vi "editDialog.vi"(0 "reference":refnum<class "NoteNode.lvclass">, 1 "insidePackageNode":bool, 5 "error in (no error)":errorcluster) -> (14 "reference out":refnum<class "NoteNode.lvclass">, 15 "changeConnection":T1, 16 "cancel":bool, 19 "error out":errorcluster)   [LabVIEW 2020, in "NoteNode.lvclass"]
doc: "Edit Dialog"
uses:
  <resource>/Framework/Providers/Open_GDS/UML/NoteNode_class/NoteNode.lvclass
  C:/Program Files (x86)/National Instruments/LabVIEW 2020/resource/Framework/Providers/Open_GDS/UML/RectangularNode_class/RectangularNode.lvclass
  C:/Program Files (x86)/National Instruments/LabVIEW 2020/resource/Framework/Providers/Open_GDS/UML/AbstractNode_class/AbstractNode.lvclass
  <resource>/Framework/Providers/Open_GDS/UML/AbstractNode_class/private/NodeConnectionStatsType.ctl
  <vilib>/Utility/miscctls.llb/LVRectTypeDef.ctl
  <vilib>/event_ctls.llb/eventvkey.ctl
  <resource>/Framework/Providers/Open_GDS/UML/ContextHelp/ContextHelp_HelpTexts.ctl
  <vilib>/Utility/miscctls.llb/LVSelectionTypeDef.ctl
  <resource>/Framework/Providers/Open_GDS/UML/MultiLineString_class/MultiLineString.lvclass
  <resource>/Framework/Providers/Open_GDS/UML/AbstractNode_class/AbstractNode.lvclass
  <resource>/Framework/Providers/Open_GDS/UML/RectangularNode_class/RectangularNode.lvclass
panel:
  in  "Underline":bool
  in  "Italic":bool
  in  "Bold":bool
  in  "Justify":u16(ring) items=["Left", "Center", "Right"]
  in  "Note color":u32(colorbox)
  in  "Help":bool
  in  "TextBox":string
  in  "connection":bool caption="Connect to Package"
  in  "OK Button":bool
  in  "Cancel Button":bool
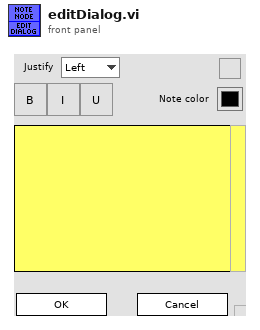
[diagram p1: front panel]
types:
  T1 = typedef "AbstractNode.lvclass/NodeConnectionStatsType.ctl" = enum16{"NA", "Connect", "DisConnect"}
  T2 = typedef "LVRectTypeDef.ctl" = cluster{"Left":i16, "Top":i16, "Right":i16, "Bottom":i16}
  T3 = cluster{"IgnoreStyleUpdate":bool, "Text":string, "Cancelled":bool, "InitSize":T2, "WidthChanged":bool}
  T4 = typedef "ContextHelp_HelpTexts.ctl" = enum16{"None(Hide)", "Default", "Help", "Welcome", "GettingStarted", "ClassDiagram_Help", "SequenceDiagram_Help", "UseCaseDiagram_Help", "BSelect", "BClass", "BInterface", "BPackage", "BNote", "BDependency", "BInheritance", "BInterfaceImplementation", "BAssociation", "BAggregation", "BCompAggregation", "BNoteConnector", "BObject", "BActionBar", "BCall", "BSystem", "BActor", "BUseCase", "BGeneralization", "BIncludes", "BExtends", "BUseCaseDiagramAssociation", "ClassRelationshipEdge editDialog_Bent Style", "ClassRelationshipEdge editDialog_RelationType", "ClassRelationshipEdge editDialog_Reverse association", "ClassRelationshipEdge editDialog_Start label", "ClassRelationshipEdge editDialog_Middle label", "ClassRelationshipEdge editDialog_End label", "UMLEditor reversedEngineering_Pathes", "ReversedEngineering StateReverseDialog_Help", "ReversedEngineering StateQueuedSettings_Help", "UMLEditor reversedEngineering_AddTopVIs", "UMLEditor reversedEngineering_AddClasses", "UMLEditor reversedEngineering_AddDirs", "UMLEditor reversedEngineering_Recursively", "UMLEditor reversedEngineering_Remove", "UMLEditor reversedEngineering_ClearList", "UMLEditor reversedEngineering_HideSubAss", "UMLEditor reversedEngineering_CreateTypes", "UMLEditor reversedEngineering_OnlyInheritance", "UMLEditor reversedEngineering_CreateApplication", "UMLEditor reversedEngineering_OK", "UMLEditor reversedEngineering_Cancel", "UMLEditor reversedEngineering_Help", "UMLEditor createWizardScriptFile_ScriptfilePath", "UMLEditor createWizardScriptFile_ClassPath", "UMLEditor createWizardScriptFile_Use", "UMLEditor createWizardScriptFile_PrivateDirName", "UMLEditor createWizardScriptFile_DirAppend", "UMLEditor createWizardScriptFile_Separator Character", "UMLEditor createWizardScriptFile_OK", "UMLEditor createWizardScriptFile_Cancel", "UMLEditor createWizardScriptFile_Help", "ClassNode editDialog_Class Name", "InterfaceNode editDialog_Class Name", "ClassNode editDialog_Attribute", "ClassNode editDialog_Methods", "InterfaceNode editDialog_Methods", "ClassNode editDialog_connection", "InterfaceNode editDialog_connection", "ClassNode editDialog_StereoType", "ClassNode editDialog_ShowAttrib", "ClassNode editDialog_ShowMethods", "ClassNode editDialog_ClassPath", "ClassNode editDialog_AddAttribute", "ClassNode editDialog_AddMethod", "InterfaceNode editDialog_AddMethod", "ClassNode AttributeGuide_AttributeName", "ClassNode AttributeGuide_Array?", "ClassNode AttributeGuide_Data Type", "ClassNode AttributeGuide_RefName", "ClassNode AttributeGuide_Preview", "ClassNode AttributeGuide_OK", "ClassNode AttributeGuide_Cancel", "ClassNode MethodGuide_Visibility", "ClassNode MethodGuide_Method Name", "ClassNode MethodGuide_Preview", "ClassNode MethodGuide_OK", "ClassNode MethodGuide_Cancel", "CallNode EditCallProperties_AllButtons", "ObjectNode EditObjectlProperties_AllButtons", "ActorNode EditActorProperties_AllButtons", "UseCaseRelationshipNode EditUseCaselProperties_AllButtons", "UseCaseNode EditUseCaselProperties_AllButtons", "SystemNode EditSystemProperties_AllButtons", "ReversedEngineering UpdateAttributes_AllButtons", "StateNode editDialog_AllButtons", "StateTransition editDialog_AllButtons", "ArrangeNodes Main_Picture", "ArrangeNodes Main_Zoom", "ArrangeNodes Main_Auto Zoom", "ArrangeNodes Main_shorten", "ArrangeNodes Main_Min Length", "ArrangeNodes Main_Max Length", "ArrangeNodes Main_increase", "ArrangeNodes Main_decrease", "ArrangeNodes Main_Shake", "ArrangeNodes Main", "BState", "BInitialState", "BFinalState", "BStateTransition", "StateDiagram_Help", "StateDiagram_PropertiesAllButtons", "ReversedEngineering StateReverseDialog_ClearStates", "ReversedEngineering StateReverseDialog_UseQueuedStateMachines", "ReversedEngineering StateReverseDialog_QueuedSettings", "ReversedEngineering StateReverseDialog_SearchForVIs", "ReversedEngineering StateReverseDialog_SearchCriteria", "OptionsDialog_ClassBasePath", "OptionsDialog_VIPath", "OptionsDialog_ApplicationPath", "OptionsDialog_WizDir", "OptionsDialog_IniFilePath", "OptionsDialog_DefineColors", "OptionsDialog_Help", "OptionsDialog_CreateTypes", "ClassRelationshipEdge editDialog_SplitWire"}
  T5 = typedef "LVSelectionTypeDef.ctl" = cluster{"Selection Start":u32, "Selection End":u32}
  T6 = typedef "NoteNode.lvclass/ObjectAttributes.ctl" = cluster{"DEFAULT_WIDTH":i32, "DEFAULT_HEIGHT":i32, "DEFAULT_COLOR":u32, "FOLD_X":i32, "FOLD_Y":i32, "color":u32, "text":refnum<class "MultiLineString.lvclass">, "pointNodes":refnum<class "AbstractNode.lvclass">[]}
  T7 = typedef "RectangularNode.lvclass/ObjectAttributes.ctl" = cluster{"bounds":T8}
  T8 = typedef "Rectangle Rectangle2D.ctl" = cluster{"x":dbl, "y":dbl, "width":dbl, "height":dbl}
  T9 = typedef "AbstractNode.lvclass/ObjectAttributes.ctl" = cluster{"parent":refnum<class "AbstractNode.lvclass">, "children":refnum<class "AbstractNode.lvclass">[], "Hidden":bool}
  T10 = typedef "MultiLineString.lvclass/JustificationType.ctl" = enum16{"LEFT", "CENTER", "RIGHT"}
  T11 = typedef "eventvkey.ctl" = enum16{"ASCII", "Enter", "Return", "Shift", "Ctrl", "Alt", "Cmd", "Opt", "Caps", "NumLock", "Clear", "Break", "Up", "Down", "Left", "Right", "Insert", "Delete", "Home", "End", "PageUp", "PageDown", "Escape", "Help", "Pause", "ScrollLock", "F1", "F2", "F3", "F4", "F5", "F6", "F7", "F8", "F9", "F10", "F11", "F12", "F13", "F14", "F15", "F16", "F17", "F18", "F19", "F20", "F21", "F22", "F23", "F24", "Play", "VolumeUp", "VolumeDown", "Mute", "Two Byte Char"}
  T12 = cluster{"Shift":bool, "Ctrl":bool, "Alt":bool, "Cmd":bool, "Opt":bool}
  T13 = typedef "ContextHelp_ShowType.ctl" = cluster{"Header":string, "Picture":picture, "Text":string}
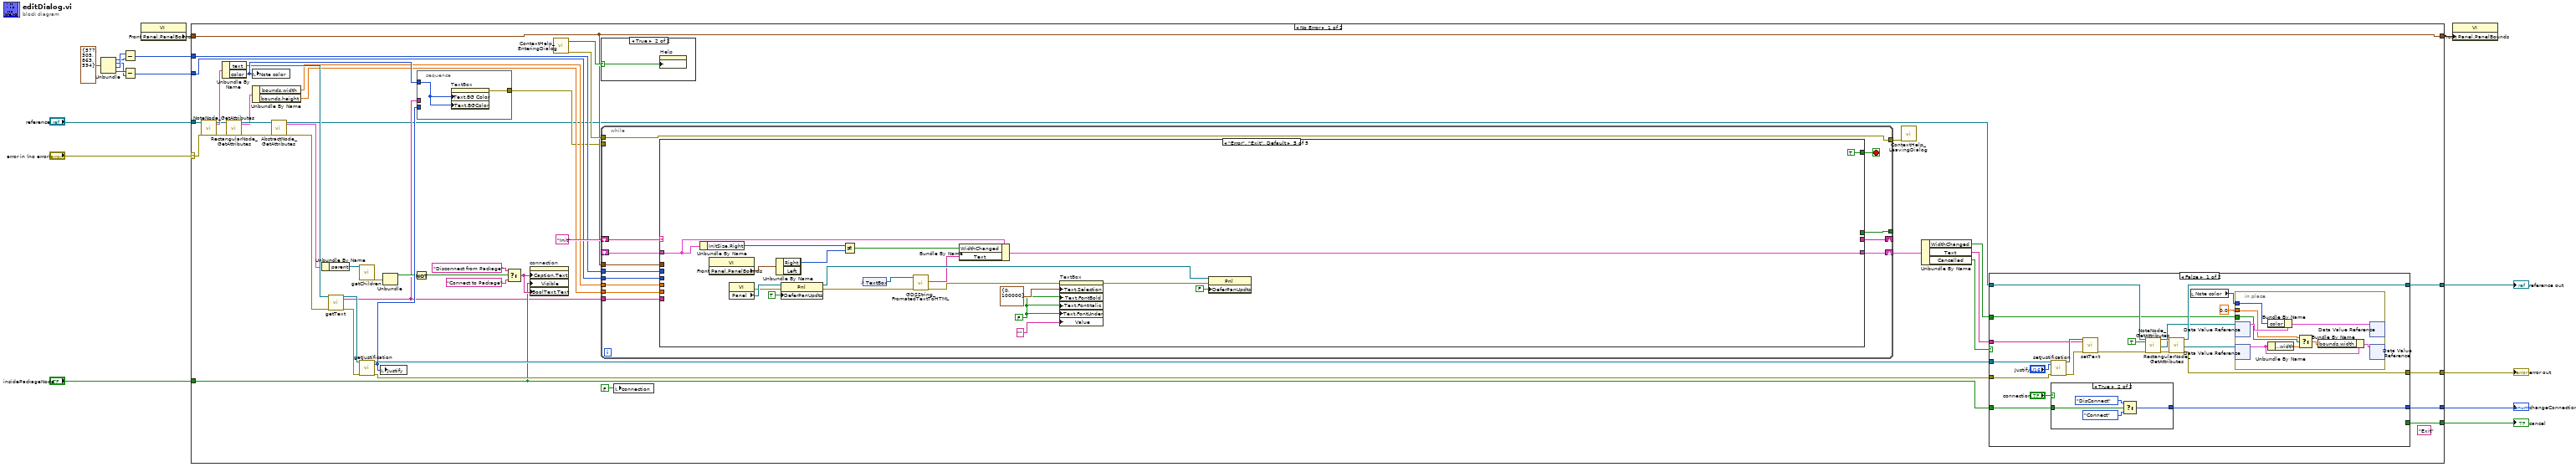
[diagram p0: block diagram]
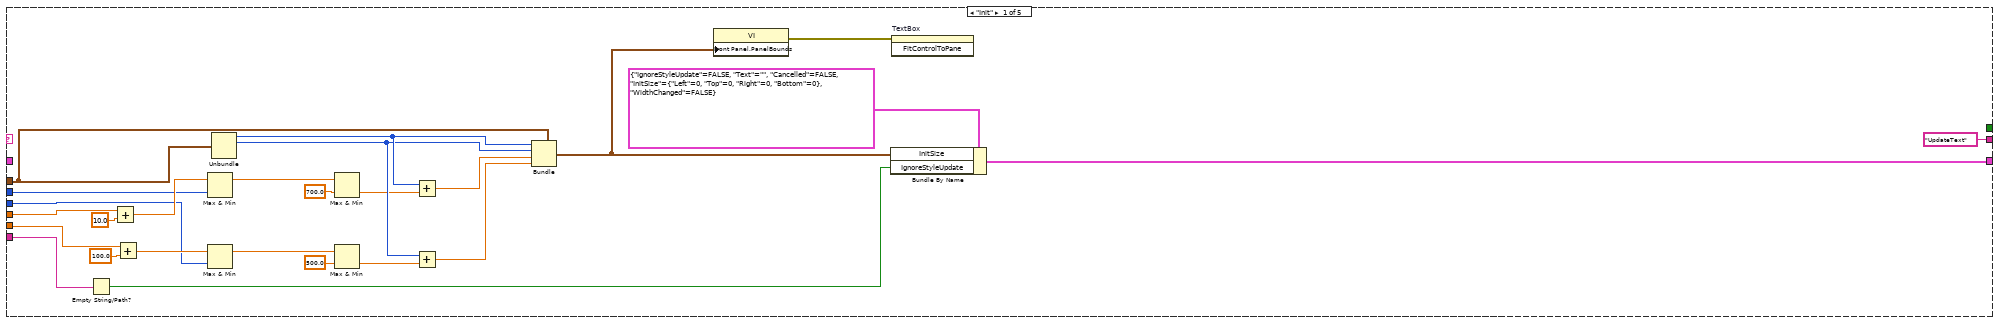
[diagram p3: hidden frame]
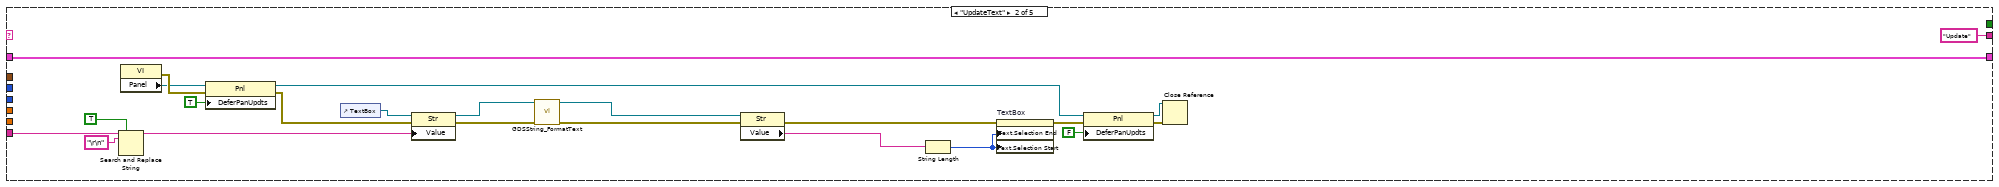
[diagram p4: hidden frame]
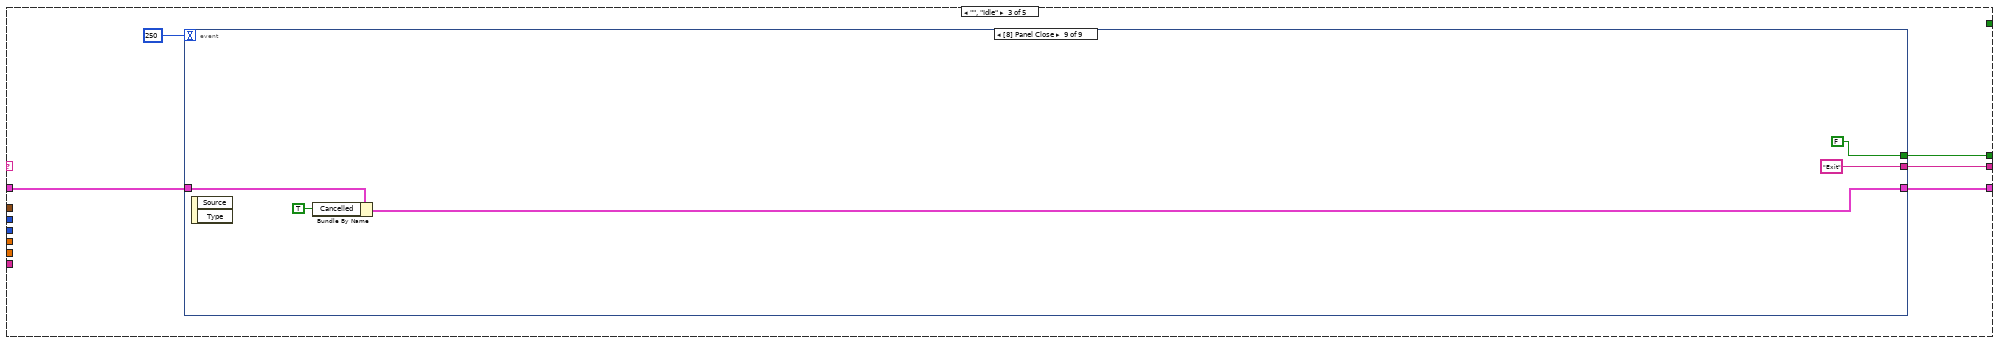
[diagram p5: hidden frame]
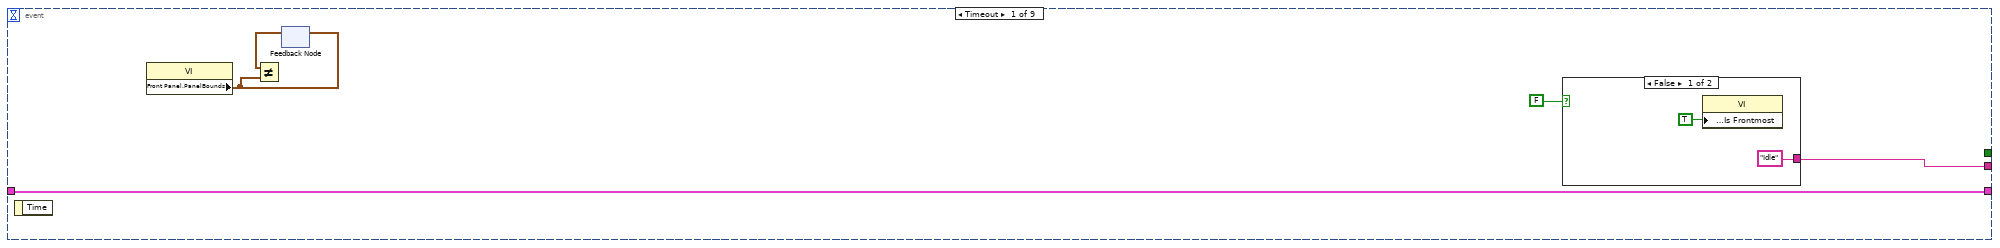
[diagram p6: hidden frame]
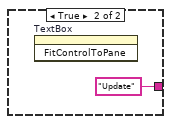
[diagram p7: hidden frame]
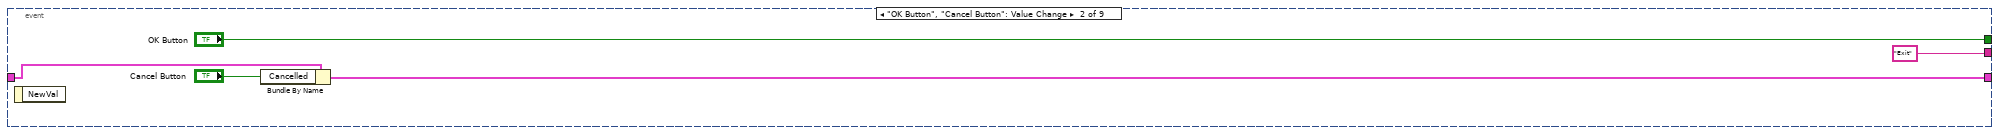
[diagram p8: hidden frame]
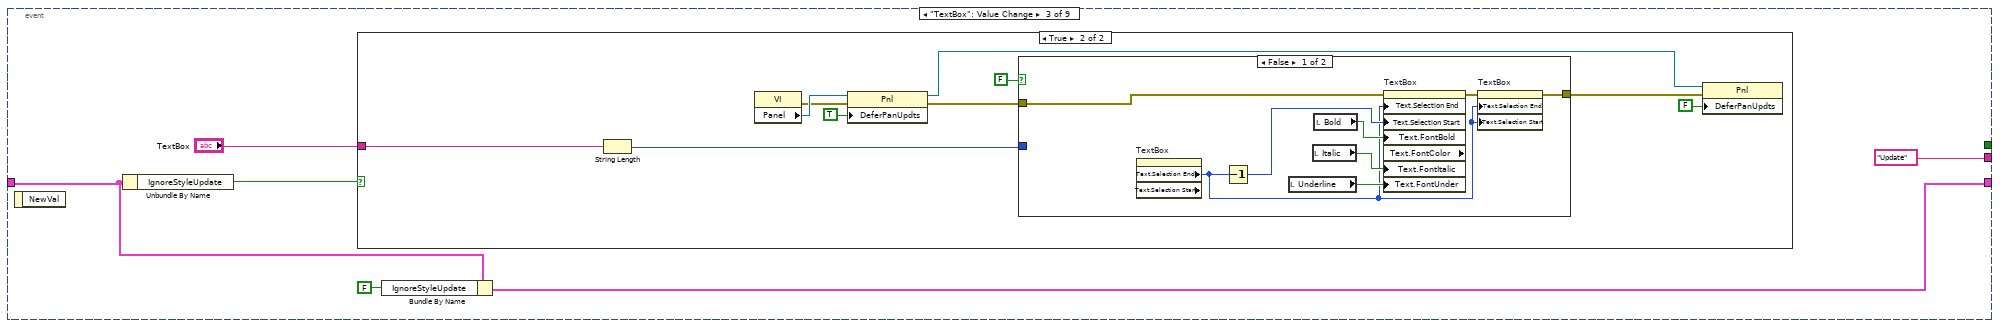
[diagram p9: hidden frame]
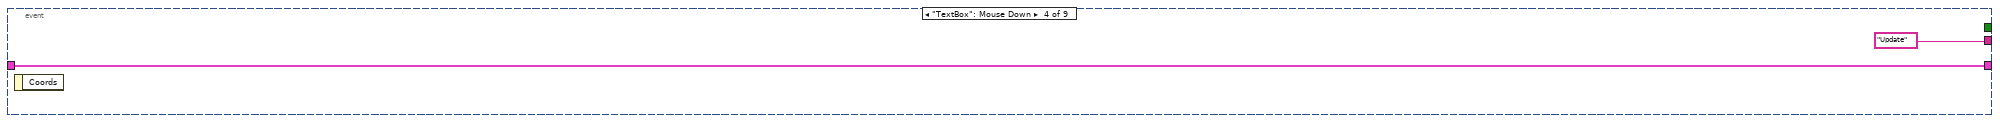
[diagram p12: hidden frame]
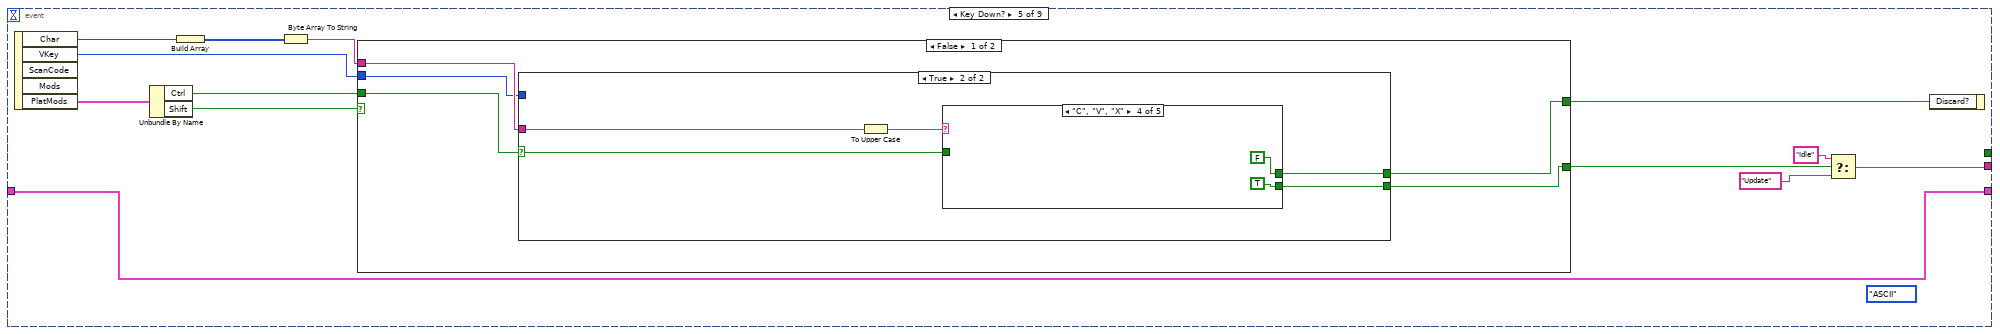
[diagram p13: hidden frame]
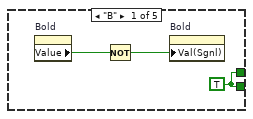
[diagram p16: hidden frame]
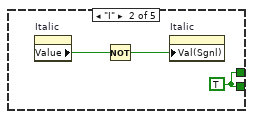
[diagram p17: hidden frame]
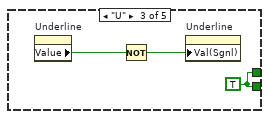
[diagram p18: hidden frame]
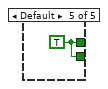
[diagram p19: hidden frame]
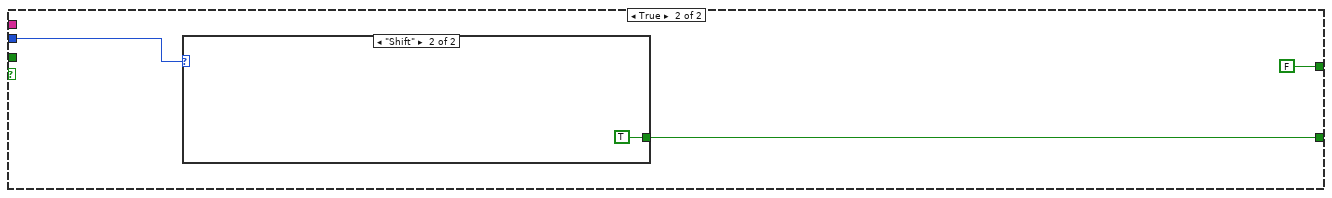
[diagram p20: hidden frame]
diagram:
  n1 = Unbundle(T2 {"Left"=577, "Top"=305, "Right"=863, "Bottom"=594} ("Front Panel Window:Panel Bounds")) -> ("Left"=w6:i16, "Top"=w4:i16, "Right"=w7:i16, "Bottom"=w5:i16)
  n2 = Subtract(x=w7, y=w6) -> (x-y=w2:i16)
  n3 = Subtract(x=w5, y=w4) -> (x-y=w1:i16)
  n4 = property class="VI"() -> ("Front Panel.PanelBounds"=w9:T2)  [unwired: 2 in, 2 out]
  n5 = case shown="No Error" "error in (no error)" {
    selector: "error in (no error)" -> [w58 w349]
    tunnel: "reference" -> [w59 w350]
    tunnel: [w62 w349] -> w14
    tunnel: [w61 w350] -> w13
    tunnel: [w56 TRUE ("Key Focus")] -> w12
    tunnel: [w47 _] -> w11
    tunnel: "insidePackageNode" -> [w39 _]
    tunnel: w9 -> [w29 w347]
    tunnel: [w29 w347] -> w3
    tunnel: w2 -> [w31 _]
    tunnel: w1 -> [w30 _]
    frame No Error {
      (unwired) "Exit"
      n6 = call <resource>:"NoteNode_GetAttributes.vi"("reference in"=w59, "error in (no error)"=w58) -> ("reference out"=w24:refnum<class "NoteNode.lvclass">, "Data"=w25:T6, "error out"=w23:errorcluster)  [unwired: 1 in, 14 out]
      n7 = Unbundle By Name(w25) -> ("text"=w57:refnum<class "MultiLineString.lvclass">, "color"=w60:u32)
      n8 = call <resource>:"RectangularNode_GetAttributes.vi"("reference in"=w24, "error in (no error)"=w23) -> ("reference out"=w22:refnum<class "NoteNode.lvclass">, "Data"=w17:T7, "error out"=w21:errorcluster)  [unwired: 14 in, 1 out]
      n9 = local write "Note color"(w60) -> ()
      n10 = Unbundle By Name(w17) -> ("bounds.width"=w33:dbl, "bounds.height"=w32:dbl)
      n11 = call <resource>:"AbstractNode_GetAttributes.vi"("reference in"=w22, "error in (no error)"=w21) -> ("reference out"=w19:refnum<class "NoteNode.lvclass">, "Data"=w18:T9, "error out"=w20:errorcluster)  [unwired: 14 in, 1 out]
      n12 = Unbundle By Name(w18) -> ("parent"=w44:refnum<class "AbstractNode.lvclass">)
      n13 = call-dynamic "getText.vi"("reference"=w57, "error in (no error)"=w20) -> ("reference out"=w52:refnum<class "MultiLineString.lvclass">, "text"=w36:string, "error out"=w51:errorcluster)  [unwired: 15 in]
      n14 = call-dynamic "getChildren.vi"("reference"=w44) -> ("error out"=w42:errorcluster)  [unwired: 15 in, 3 out]
      n15 = call <resource>:"getJustification.vi"("reference"=w52, "error in (no error)"=w51) -> ("reference out"=w49:refnum<class "MultiLineString.lvclass">, "justification"=w48:T10, "error out"=w50:errorcluster)  [unwired: 15 out]
      n16 = local write "Justify"(w48) -> ()
      n17 = Unbundle(w42) -> ("status"=w43:bool)  [unwired: 2 out]
      n18 = Not(x=w43) -> (.not. x?=w45:bool)
      n19 = stacked-sequence {
        tunnel: w60 -> [w346]
        tunnel: w36 -> [_]
        tunnel: w48 -> [_]
        tunnel: [w345] -> w28
        frame #0 {
          n20 = property on="TextBox" class="Str"("Text.BG Color"=w346, "Text.BGColor"=w346) -> (error out=w345:errorcluster)  [unwired: 2 in, 1 out]
        }
      }
      n21 = Select(t="Disconnect from Package", s=w45, f="Connect to Package") -> (s? t:f=w46:string)
      n22 = property on="connection" class="Bool (strict)"("Caption.Text"=w46, "Visible"=w39, "BoolText.Text"=w46) -> ()  [unwired: 2 in, 2 out]
      n23 = call <resource>:"ContextHelp_EnteringDialog.vi"() -> ("HelpStatus"=w53:bool, "error out"=w54:errorcluster)  [unwired: 3 in, 15 out]
      n24 = case shown="True" w53 {
        selector: w53 -> [_ w63]
        frame False {
        }
        frame True {
          n25 = property on="Help" class="Bool (strict)"("Value (Signaling)"=w63) -> ()  [unwired: 2 in, 2 out]
        }
      }
      n26 = while {
        tunnel: [w76] -> _
        tunnel: [w74] -> w55
        tunnel: w54 -> [w74]
        shift-right: [w71] -> _
        shift-left: "Init" -> [w73]
        tunnel: w36 -> [w72]
        shift-right: [w70] -> w35
        shift-left: _ -> [w69]
        tunnel: w33 -> [w68]
        tunnel: w32 -> [w67]
        tunnel: w31 -> [w66]
        tunnel: w30 -> [w65]
        tunnel: w29 -> [w64]
        tunnel: w28 -> [_]
        stop <- w75 stop-if-true
        n27 = case shown="\"Error\", \"Exit\", Default" w73 {
          tunnel: [_ _ w130 _ _] -> w76
          tunnel: [_ _ _ _ TRUE ("Key Focus")] -> w75
          tunnel: w72 -> [w82 w107 _ _ _]
          tunnel: ["UpdateText" "Update" w128 _ _] -> w71
          tunnel: [w79 w116 w126 w239 w292] -> w70
          tunnel: w69 -> [_ w116 w127 w240 w291]
          tunnel: w68 -> [w101 _ _ _ _]
          tunnel: w67 -> [w100 _ _ _ _]
          tunnel: w66 -> [w95 _ _ _ _]
          tunnel: w65 -> [w94 _ _ _ _]
          tunnel: w64 -> [w93 _ _ _ _]
          frame "Init" {
            n28 = Empty String/Path?(string/path=w82) -> (empty?=w80:bool)
            n29 = Add(x=w101, y=10.0) -> (x+y=w97:dbl)
            n30 = Add(x=w100, y=100.0) -> (x+y=w96:dbl)
            n31 = Max & Min(x=w97, y=w95) -> (max(x,y)=w86:dbl)  [unwired: 1 out]
            n32 = Max & Min(x=w96, y=w94) -> (max(x,y)=w88:dbl)  [unwired: 1 out]
            n33 = Unbundle(w93) -> ("Left"=w92:i16, "Top"=w90:i16)  [unwired: 2 out]
            n34 = Max & Min(x=w86, y=700.0) -> (min(x,y)=w85:dbl)  [unwired: 1 out]
            n35 = Max & Min(x=w88, y=500.0) -> (min(x,y)=w87:dbl)  [unwired: 1 out]
            n36 = Add(x=w92, y=w85) -> (x+y=w91:dbl)
            n37 = Add(x=w90, y=w87) -> (x+y=w89:dbl)
            n38 = Bundle(cluster=w93, "Left"=w92, "Top"=w90, "Right"=w91, "Bottom"=w89) -> (w77:T2)
            n39 = property class="VI"("Front Panel.PanelBounds"=w77) -> (error out=w78:errorcluster)  [unwired: 2 in, 1 out]
            n40 = Bundle By Name(cluster=T3 {"IgnoreStyleUpdate"=FALSE, "Text"="", "Cancelled"=FALSE, "InitSize"={"Left"=0, "Top"=0, "Right"=0, "Bottom"=0}, "WidthChanged"=FALSE} ("State"), "InitSize"=w77, "IgnoreStyleUpdate"=w80) -> (w79:T3)
            n41 = invoke on="TextBox" class="Str" method="FitControlToPane"(error in=w78) -> ()  [unwired: 2 in, 3 out]
          }
          frame "UpdateText" {
            n42 = Search and Replace String(replace all?=TRUE ("replace all? (F)"), input string=w107, search string="\r\n") -> (result string=w106:string)  [unwired: 5 in, 3 out]
            n43 = property class="VI"() -> (error out=w121:errorcluster, "Panel"=w119:refnum<vi>)  [unwired: 2 in, 1 out]
            n44 = property class="Pnl"(reference=w119, error in=w121, "DeferPanUpdts"=TRUE ("Defer Panel Updates")) -> (reference out=w123:refnum<vi>, error out=w122:errorcluster)
            n45 = control-ref of="TextBox"() -> (w115:refnum<vi>)
            n46 = property on="Property Node" class="Str"(reference=w115, error in=w122, "Value"=w106) -> (reference out=w117:refnum<vi>, error out=w118:errorcluster)
            n47 = call <resource>:"GDSString_FormatText.vi"("TextIn"=w117, "error in"=w118) -> ("TextOut"=w114:refnum<vi>, "error out"=w113:errorcluster)  [unwired: 16 in]
            n48 = property on="Property Node" class="Str"(reference=w114, error in=w113) -> (error out=w112:errorcluster, "Value"=w111:string)  [unwired: 1 out]
            n49 = String Length(string=w111) -> (length=w108:i32)
            n50 = property on="TextBox" class="Str"(error in=w112, "Text.Selection End"=w108, "Text.Selection Start"=w108) -> (error out=w110:errorcluster)  [unwired: 1 in, 1 out]
            n51 = property class="Pnl"(reference=w123, error in=w110, "DeferPanUpdts"=FALSE ("Defer Panel Updates")) -> (reference out=w124:refnum<vi>, error out=w105:errorcluster)
            n52 = Close Reference(reference=w124, error in (no error)=w105) -> ()  [unwired: 1 out]
          }
          frame "", "Idle" {
            n53 = event shown="[8] Panel Close" {
              selector: _ -> [_ _ _ _ _ _ _ _ _]
              dyn-events: _ -> [_ _ _ _ _ _ _ _ _]
              timeout: 250 -> [_ _ _ _ _ _ _ _ _]
              tunnel: [_ "OK Button" _ _ _ _ _ _ FALSE ("OK Button")] -> w130
              tunnel: [w132 "Exit" "Update" "Update" w171 _ "Update" "Idle" "Exit"] -> w128
              tunnel: w127 -> [w135 w141 w146 w170 w183 w212 w218 w227 w236]
              tunnel: [w135 w140 w147 w170 w183 w212 w217 w227 w235] -> w126
              event Timeout {
                n54 = event-data() -> ()  [unwired: 2 out]
                n55 = property class="VI"() -> ("Front Panel.PanelBounds"=w134:T2)  [unwired: 2 in, 2 out]
                n56 = feedback-in #1(w134) -> ()
                n57 = feedback #1() -> (w133:T2)  [unwired: 1 in]
                n58 = Not Equal?(x=w133, y=w134) -> ()  [unwired: 1 out]
                n59 = case shown="False" FALSE {
                  tunnel: ["Idle" "Update"] -> w132
                  frame False {
                    n60 = property class="VI"("Front Panel Window:Is Frontmost"=TRUE) -> ()  [unwired: 2 in, 2 out]
                  }
                  frame True {
                    n61 = invoke on="TextBox" class="Str" method="FitControlToPane"() -> ()  [unwired: 3 in, 3 out]
                  }
                }
              }
              event "OK Button", "Cancel Button": Value Change {
                n62 = event-data() -> ()  [unwired: 2 out]
                n63 = Bundle By Name(cluster=w141, "Cancelled"="Cancel Button") -> (w140:T3)
              }
              event "TextBox": Value Change {
                n64 = event-data() -> ()  [unwired: 2 out]
                n65 = Unbundle By Name(w146) -> ("IgnoreStyleUpdate"=w149:bool)
                n66 = case shown="True" w149 {
                  tunnel: "TextBox" -> [_ w151]
                  frame False {
                  }
                  frame True {
                    n67 = String Length(string=w151) -> (length=w152:i32)
                    n68 = property class="VI"() -> (error out=w157:errorcluster, "Panel"=w159:refnum<vi>)  [unwired: 2 in, 1 out]
                    n69 = property class="Pnl"(reference=w159, error in=w157, "DeferPanUpdts"=TRUE ("Defer Panel Updates")) -> (reference out=w155:refnum<vi>, error out=w154:errorcluster)
                    n70 = case shown="False" FALSE {
                      tunnel: w152 -> [_ _]
                      tunnel: w154 -> [w166 w168]
                      tunnel: [w164 w168] -> w153
                      frame False {
                        n71 = property on="TextBox" class="Str" props=["Text", "Selection End", "Text", "Selection Start"]() -> ("Text.Selection End"=w160:u32)  [unwired: 2 in, 3 out]
                        n72 = Decrement(x=w160) -> (x-1=w167:u32)
                        n73 = local read "Underline"() -> (w161:bool)
                        n74 = local read "Italic"() -> (w162:bool)
                        n75 = local read "Bold"() -> (w163:bool)
                        n76 = property on="TextBox" class="Str" props=["Text", "Selection End", "Text", "Selection Start", "Text", "FontBold", "Text", "FontColor", "Text", "FontItalic", "Text", "FontUnder"](error in=w166, "Text.Selection End"=w160, "Text.Selection Start"=w167, "Text.FontBold"=w163, "Text.FontItalic"=w162, "Text.FontUnder"=w161) -> (error out=w165:errorcluster)  [unwired: 1 in, 2 out]
                        n77 = property on="TextBox" class="Str"(error in=w165, "Text.Selection End"=w160, "Text.Selection Start"=w160) -> (error out=w164:errorcluster)  [unwired: 1 in, 1 out]
                      }
                      frame True {
                      }
                    }
                    n78 = property class="Pnl"(reference=w155, error in=w153, "DeferPanUpdts"=FALSE ("Defer Panel Updates")) -> ()  [unwired: 2 out]
                  }
                }
                n79 = Bundle By Name(cluster=w146, "IgnoreStyleUpdate"=FALSE ("NewType")) -> (w147:T3)
              }
              event "TextBox": Mouse Down {
                n80 = event-data() -> ()  [unwired: 2 out]
              }
              event Key Down? {
                (unwired) eventvkey."ASCII" ("VKey")
                n81 = event-data() -> ("Char"=w178:i16, "VKey"=w177:T11, "PlatMods"=w176:T12)  [unwired: 3 out]
                n82 = Unbundle By Name(w176) -> ("Ctrl"=w180:bool, "Shift"=w179:bool)
                n83 = Build Array(w178) -> (w182:i16[])
                n84 = Byte Array To String(unsigned byte array=w182) -> (string=w181:string)
                n85 = case shown="False" w179 {
                  tunnel: w180 -> [w188 _]
                  tunnel: w181 -> [w187 _]
                  tunnel: [w186 FALSE ("Discard?")] -> w175
                  tunnel: [w185 w209] -> w174
                  tunnel: w177 -> [w184 w207]
                  frame False {
                    n86 = case shown="True" w188 {
                      selector: w188 -> [_ w192]
                      tunnel: w187 -> [_ w194]
                      tunnel: [_ w191] -> w186
                      tunnel: [_ w190] -> w185
                      tunnel: w184 -> [w189 _]
                      frame False {
                        n87 = case shown="\"ASCII\", Default" w189 {
                          frame "ASCII", Default {
                          }
                          frame "Home" {
                          }
                        }
                      }
                      frame True {
                        n88 = To Upper Case(1:w194) -> (0:w193:string)
                        n89 = case shown="\"C\", \"V\", \"X\"" w193 {
                          tunnel: w192 -> [_ _ _ _ _]
                          tunnel: [w195 w198 w201 FALSE ("Discard?") w206] -> w191
                          tunnel: [w195 w198 w201 TRUE ("Discard?") w206] -> w190
                          frame "B" {
                            w195 = TRUE ("Discard?")
                            n90 = property on="Bold" class="Bool (strict)"() -> ("Value"=w197:bool)  [unwired: 2 in, 2 out]
                            n91 = Not(x=w197) -> (.not. x?=w196:bool)
                            n92 = property on="Bold" class="Bool (strict)"("Val(Sgnl)"=w196) -> ()  [unwired: 2 in, 2 out]
                          }
                          frame "I" {
                            w198 = TRUE ("Discard?")
                            n93 = property on="Italic" class="Bool (strict)"() -> ("Value"=w200:bool)  [unwired: 2 in, 2 out]
                            n94 = Not(x=w200) -> (.not. x?=w199:bool)
                            n95 = property on="Italic" class="Bool (strict)"("Val(Sgnl)"=w199) -> ()  [unwired: 2 in, 2 out]
                          }
                          frame "U" {
                            w201 = TRUE ("Discard?")
                            n96 = property on="Underline" class="Bool (strict)"() -> ("Value"=w203:bool)  [unwired: 2 in, 2 out]
                            n97 = Not(x=w203) -> (.not. x?=w202:bool)
                            n98 = property on="Underline" class="Bool (strict)"("Val(Sgnl)"=w202) -> ()  [unwired: 2 in, 2 out]
                          }
                          frame "C", "V", "X" {
                          }
                          frame Default {
                            w206 = TRUE
                          }
                        }
                      }
                    }
                  }
                  frame True {
                    n99 = case shown="\"Shift\"" w207 {
                      tunnel: [_ TRUE] -> w209
                      frame Default {
                      }
                      frame "Shift" {
                      }
                    }
                  }
                }
                n100 = Select(t="Idle", s=w174, f="Update") -> (s? t:f=w171:string)
                n101 = event-data("Discard?"=w175) -> ()  [unwired: 1 in, 1 out]
              }
              event "Note color": Value Change {
                (unwired) "Idle"
                n102 = event-data() -> ()  [unwired: 2 out]
                n103 = property on="TextBox" class="Str"("Text.BG Color"="Note color", "Text.BGColor"="Note color") -> ()  [unwired: 2 in, 2 out]
              }
              event "Bold", "Italic", "Underline": Value Change {
                (unwired) TRUE ("Data Changed?")
                n104 = event-data() -> ()  [unwired: 2 out]
                n105 = property on="TextBox" class="Str"() -> ("Text.Selection End"=w223:u32, "Text.Selection Start"=w222:u32)  [unwired: 2 in, 2 out]
                n106 = local read "TextBox"() -> (w221:string)
                n107 = String Length(string=w221) -> (length=w220:i32)
                n108 = Equal?(x=w223, y=w222) -> (x = y?=w219:bool)
                n109 = Bundle By Name(cluster=w218, "IgnoreStyleUpdate"=w219) -> (w217:T3)
                n110 = case shown="False" w219 {
                  tunnel: "Bold" -> [w226 _]
                  tunnel: w220 -> [_ _]
                  tunnel: "Italic" -> [w225 _]
                  tunnel: "Underline" -> [w224 _]
                  frame False {
                    n111 = property on="TextBox" class="Str"("Text.FontUnder"=w224) -> ()  [unwired: 2 in, 2 out]
                    n112 = property on="TextBox" class="Str"("Text.FontBold"=w226) -> ()  [unwired: 2 in, 2 out]
                    n113 = property on="TextBox" class="Str"("Text.FontItalic"=w225) -> ()  [unwired: 2 in, 2 out]
                  }
                  frame True {
                  }
                }
              }
              event "Help": Value Change {
                n114 = event-data() -> ()  [unwired: 2 out]
                n115 = case shown="True" "Help" {
                  tunnel: [ContextHelp_HelpTexts."None(Hide)" ("HelpText") ContextHelp_HelpTexts."BNote" ("HelpText")] -> w230
                  frame False {
                  }
                  frame True {
                  }
                }
                n116 = call <resource>:"ContextHelp_HelpTexts.vi"("HelpText (enum or string)"=w230) -> ("HelpOut"=w231:T13)  [unwired: 18 out]
                n117 = call <resource>:"ContextHelp_SendMessageToPopUp.vi"("PopUpMessage"=w231) -> ()  [unwired: 2 in, 17 out]
              }
              event Panel Close {
                n118 = event-data() -> ()  [unwired: 3 out]
                n119 = Bundle By Name(cluster=w236, "Cancelled"=TRUE ("Key Focus")) -> (w235:T3)
              }
            }
          }
          frame "Update" {
            n120 = Unbundle By Name(w240) -> ("IgnoreStyleUpdate"=w241:bool)
            n121 = case shown="False" w241 {
              tunnel: [w249 _] -> w243
              tunnel: w240 -> [w245 w286]
              tunnel: [w245 w286] -> w239
              frame False {
                n122 = property on="TextBox" class="Str"() -> (error out=w250:errorcluster, "Text.Selection End"=w246:u32, "Text.Selection Start"=w247:u32)  [unwired: 2 in, 1 out]
                n123 = Not Equal?(x=w246, y=w247) -> (x != y?=w248:bool)
                n124 = property class="VI"(error in=w250) -> (error out=w257:errorcluster, "Panel"=w259:refnum<vi>)  [unwired: 1 in, 1 out]
                n125 = property class="Pnl"(reference=w259, error in=w257, "DeferPanUpdts"=TRUE ("Defer Panel Updates")) -> (reference out=w252:refnum<vi>, error out=w244:errorcluster)
                n126 = case shown="False" w248 {
                  tunnel: [w264 w283] -> w255
                  tunnel: [w265 w284] -> w254
                  tunnel: [w266 w285] -> w253
                  tunnel: w247 -> [w260 w279]
                  tunnel: w244 -> [w263 w281]
                  tunnel: [w261 w282] -> w251
                  tunnel: w246 -> [_ w278]
                  frame False {
                    n127 = case shown="Default" w260 {
                      selector: w260 -> [_ w271]
                      tunnel: [w267 w276] -> w266
                      tunnel: [w268 w275] -> w265
                      tunnel: [w269 w274] -> w264
                      tunnel: w263 -> [w270 w273]
                      tunnel: [w270 w272] -> w262
                      frame 0 {
                        n128 = local read "Underline"() -> (w267:bool)
                        n129 = local read "Bold"() -> (w269:bool)
                        n130 = local read "Italic"() -> (w268:bool)
                      }
                      frame Default {
                        n131 = Decrement(x=w271) -> (x-1=w277:u32)
                        n132 = property on="TextBox" class="Str" props=["Text", "Selection End", "Text", "Selection Start", "Text", "FontBold", "Text", "FontColor", "Text", "FontItalic", "Text", "FontUnder"](error in=w273, "Text.Selection End"=w271, "Text.Selection Start"=w277) -> (error out=w272:errorcluster, "Text.FontBold"=w274:bool, "Text.FontItalic"=w275:bool, "Text.FontUnder"=w276:bool)  [unwired: 1 in, 2 out]
                      }
                    }
                    n133 = property on="TextBox" class="Str"(error in=w262, "Text.Selection End"=w260, "Text.Selection Start"=w260) -> (error out=w261:errorcluster)  [unwired: 1 in, 1 out]
                  }
                  frame True {
                    n134 = property on="TextBox" class="Str"(error in=w281, "Text.Selection End"=w278, "Text.Selection Start"=w279) -> (error out=w280:errorcluster)  [unwired: 1 in, 1 out]
                    n135 = property on="TextBox" class="Str" props=["Text", "FontBold", "Text", "FontColor", "Text", "FontItalic", "Text", "FontUnder"](error in=w280) -> (error out=w282:errorcluster, "Text.FontBold"=w283:bool, "Text.FontItalic"=w284:bool, "Text.FontUnder"=w285:bool)  [unwired: 1 in, 2 out]
                  }
                }
                n136 = local write "Bold"(w255) -> ()
                n137 = local write "Italic"(w254) -> ()
                n138 = local write "Underline"(w253) -> ()
                n139 = property class="Pnl"(reference=w252, error in=w251, "DeferPanUpdts"=FALSE ("Defer Panel Updates")) -> (error out=w249:errorcluster)  [unwired: 1 out]
              }
              frame True {
              }
            }
            n140 = property on="TextBox" class="Str"(error in=w243, "Key Focus"=TRUE) -> ()  [unwired: 1 in, 2 out]
          }
          frame "Error", "Exit", Default {
            w299 = FALSE ("Text.Font:Bold")
            n141 = Unbundle By Name(w291) -> ("InitSize.Right"=w288:i16)
            n142 = property class="VI"() -> ("Front Panel.PanelBounds"=w290:T2)  [unwired: 2 in, 2 out]
            n143 = property class="VI"() -> (error out=w303:errorcluster, "Panel"=w305:refnum<vi>)  [unwired: 2 in, 1 out]
            n144 = Unbundle By Name(w290) -> ("Right"=w289:i16)  [unwired: 1 out]
            n145 = property class="Pnl"(reference=w305, error in=w303, "DeferPanUpdts"=TRUE ("Defer Panel Updates")) -> (reference out=w301:refnum<vi>, error out=w294:errorcluster)
            n146 = Not Equal?(x=w288, y=w289) -> (x != y?=w287:bool)
            n147 = control-ref of="TextBox"() -> (w296:refnum<vi>)
            n148 = call <resource>:"GDSString_FromatedTextToHTML.vi"("error in (no error)"=w294, "FormattedStringIn"=w296) -> ("error out"=w293:errorcluster, "TextOut"=w295:string)  [unwired: 7 in, 1 out]
            n149 = Bundle By Name(cluster=w291, "WidthChanged"=w287, "Text"=w295) -> (w292:T3)
            n150 = property on="TextBox" class="Str"(error in=w293, "Text.Selection"=T5 {"Selection Start"=0, "Selection End"=100000}, "Text.FontBold"=w299, "Text.FontItalic"=w299, "Text.FontUnder"=w299, "Value"="" ("TextBox")) -> (error out=w297:errorcluster)  [unwired: 1 in, 1 out]
            n151 = property class="Pnl"(reference=w301, error in=w297, "DeferPanUpdts"=FALSE ("Defer Panel Updates")) -> ()  [unwired: 2 out]
          }
        }
      }
      n152 = local write "connection"(FALSE ("connection")) -> ()
      n153 = call <resource>:"ContextHelp_LeavingDialog.vi"("error in (no error)"=w55) -> ()  [unwired: 2 in, 17 out]
      n154 = Unbundle By Name(w35) -> ("WidthChanged"=w26:bool, "Text"=w34:string, "Cancelled"=w27:bool)
      n155 = case shown="False" w27 {
        tunnel: [w327 w343] -> w62
        tunnel: [w326 w344] -> w61
        tunnel: w19 -> [w325 w344]
        tunnel: w49 -> [w320 _]
        tunnel: w50 -> [w323 w343]
        tunnel: [_ TRUE ("Key Focus")] -> w56
        tunnel: [w317 _] -> w47
        tunnel: w39 -> [w316 _]
        tunnel: w34 -> [w315 _]
        tunnel: w26 -> [w308 _]
        frame False {
          n156 = call <resource>:"setJustification.vi"("reference"=w320, "justification"="Justify", "error in (no error)"=w323) -> ("reference out"=w321:refnum<class "MultiLineString.lvclass">, "error out"=w322:errorcluster)  [unwired: 15 out]
          n157 = case shown="True" "connection" {
            tunnel: [enum16{"NA", "Connect", "DisConnect"}."NA" ("changeConnection") w340] -> w317
            tunnel: w316 -> [_ w341]
            frame False {
            }
            frame True {
              n158 = Select(t=enum16{"NA", "Connect", "DisConnect"}."DisConnect" ("changeConnection"), s=w341, f=enum16{"NA", "Connect", "DisConnect"}."Connect" ("changeConnection")) -> (s? t:f=w340:enum16{"NA", "Connect", "DisConnect"})
            }
          }
          n159 = call-dynamic "setText.vi"("reference"=w321, "text"=w315, "error in (no error)"=w322) -> ("error out"=w324:errorcluster)  [unwired: 15 in, 1 out]
          n160 = call <resource>:"NoteNode_GetAttributes.vi"("reference in"=w325, "OnlyGetDvrReference(False)"=TRUE, "error in (no error)"=w324) -> ("reference out"=w313:refnum<class "NoteNode.lvclass">, "DataRef"=w311:refnum<data-value>, "error out"=w312:errorcluster)  [unwired: 13 in, 1 out]
          n161 = call <resource>:"RectangularNode_GetAttributes.vi"("reference in"=w313, "error in (no error)"=w312) -> ("reference out"=w326:refnum<class "NoteNode.lvclass">, "DataRef"=w310:refnum<data-value>, "error out"=w327:errorcluster)  [unwired: 14 in, 1 out]
          n162 = local read "Note color"() -> (w309:u32)
          n163 = in-place {
            in-place-border: w309 -> [w335]
            in-place-border: w308 -> [w329]
            in-place-border: 0.0 ("t") -> [w328]
            n164 = in-place-dvr #2(w311) -> (w336:T6)  [unwired: 1 out]
            n165 = in-place-dvr #3(w310) -> (w333:T7)  [unwired: 1 out]
            n166 = Unbundle By Name(w333) -> ("bounds.width"=w332:dbl)
            n167 = Bundle By Name(cluster=w336, "color"=w335) -> (w334:T6)
            n168 = Select(t=w328, s=w329, f=w332) -> (s? t:f=w331:dbl)
            n169 = Bundle By Name(cluster=w333, "bounds.width"=w331) -> (w330:T7)
            n170 = in-place-dvr #2(w334) -> ()  [unwired: 2 out]
            n171 = in-place-dvr #3(w330) -> ()  [unwired: 2 out]
          }
        }
        frame True {
        }
      }
    }
    frame Error {
    }
  }
  "reference out" <- w13
  "error out" <- w14
  "changeConnection" <- w11
  "cancel" <- w12
  n172 = property class="VI"("Front Panel.PanelBounds"=w3) -> ()  [unwired: 2 in, 2 out]
